vi "AutoHelperDelayedAction_Example.vi"() -> ()   [LabVIEW 2019]
uses:
  <vilib>/Rock Robotics/WPI/ThirdParty/JAS_Junk/TrajLib/VI/Util_GetTime_U32.vi
  <vilib>/Rock Robotics/WPI/ThirdParty/JAS_Junk/TrajLib/VI/DigSeqLogic_Edge_On.vi
  <vilib>/Rock Robotics/WPI/ThirdParty/JAS_Junk/TrajLib/Timer_New.vi
  <vilib>/Rock Robotics/WPI/ThirdParty/JAS_Junk/TrajLib/DigSeqLogic_SR_FlipFlop.vi
  <vilib>/Rock Robotics/WPI/ThirdParty/JAS_Junk/TrajLib/DigSeqLogic_Off_Delay.vi
  <vilib>/Rock Robotics/WPI/ThirdParty/JAS_Junk/TrajLib/VI/Util_GetTime_U64.vi
  <vilib>/Utility/semaphor.llb/Obtain Semaphore Reference.vi
  <vilib>/Rock Robotics/WPI/ThirdParty/JAS_Junk/TrajLib/Timer_Reset.vi
  <vilib>/Rock Robotics/WPI/ThirdParty/JAS_Junk/TrajLib/Timer_Start.vi
  <vilib>/Rock Robotics/WPI/ThirdParty/JAS_Junk/TrajLib/Timer_HasPeriodPassedOnce.vi
  <vilib>/Rock Robotics/WPI/ThirdParty/JAS_Junk/TrajLib/Timer_Stop.vi
  <vilib>/Rock Robotics/WPI/ThirdParty/JAS_Junk/TrajLib/VI/Timer_Restart.vi
  <vilib>/Rock Robotics/WPI/ThirdParty/JAS_Junk/TrajLib/Trajectory_Library.lvlib
panel:
  out "Delayed Action Pulse":bool
  out "Remaining\nTime":dbl format="%12.2f"
  in  "Step Start":bool
  out "Waveform Chart":cluster{i16, i16, i16}(graph)
  out "Delayed Action":bool
  out "Step Start FB":bool
  in  "Delay (sec)":dbl=4.0
  # "AUTO HELPER DELAYED ACTION"
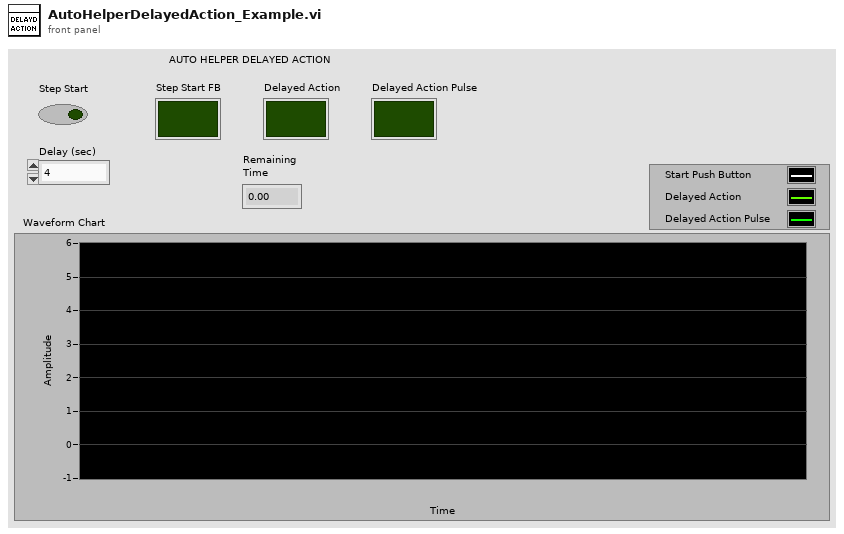
[diagram p1: front panel]
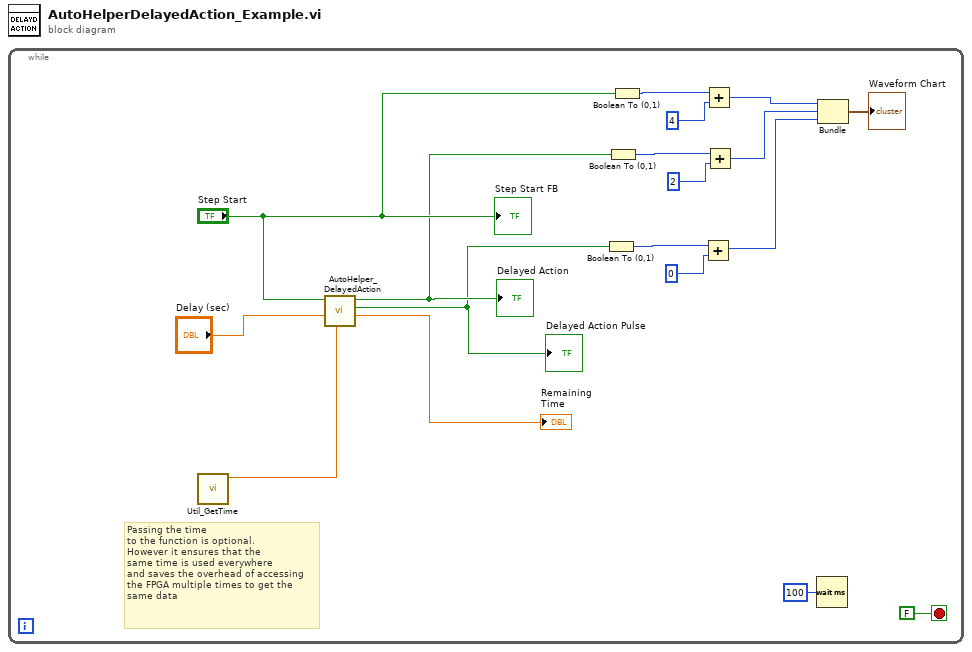
[diagram p0: block diagram]
diagram:
  n1 = while {
    stop <- FALSE stop-if-true
    # "Passing the time\nto the function is optional.\nHowever it ensures that the\nsame time is used everywhere\nand saves the overhead of accessing\nthe FPGA multiple times to get the\nsame data"
    n2 = call <vilib>:"Util_GetTime.vi"() -> ("FPGA_Time_Seconds"=w12:dbl)  [unwired: 9 in, 2 out]
    n3 = call <vilib>:"AutoHelper_DelayedAction.vi"("Pass_Through_Time"=w12, "Delay Time Sec"="Delay (sec)", "New Step"="Step Start") -> ("Remaining Delay Time Sec"=→"Remaining\nTime":dbl, "Delayed Action Pulse"=w3:bool, "Delayed Action"=w10:bool)  [unwired: 4 in, 2 out]
    "Delayed Action" <- w10
    "Delayed Action Pulse" <- w3
    n4 = Boolean To (0,1)(Boolean=w3) -> (0, 1=w4:i16)
    n5 = Boolean To (0,1)(Boolean=w10) -> (0, 1=w6:i16)
    n6 = Boolean To (0,1)(Boolean="Step Start") -> (0, 1=w15:i16)
    n7 = Add(x=w4, y=i16 0) -> (x+y=w2:i16)
    n8 = Add(x=w15, y=i16 4) -> (x+y=w14:i16)
    n9 = Add(x=w6, y=i16 2) -> (x+y=w7:i16)
    n10 = Wait (ms)(milliseconds to wait=u32 100) -> ()  [unwired: 1 out]
    n11 = Bundle(w14, w7, w2) -> (→"Waveform Chart":cluster{i16, i16, i16})  [unwired: 1 in]
    "Step Start FB" <- "Step Start"
  }
